vi "[ce] Error Handler.vi"(6 "nesting level":i32, 8 "error in":errorcluster, 9 "error reason":string, 10 "error location":string, 11 "error code":i32) -> (0 "error out":errorcluster, 3 "error":bool)   [LabVIEW 2021]
doc: "The VI builds standard error cluster on the base of input parameters and returns it in <B>error out</B> cluster. If <B>error in</B> indicates an error or <B>error code</B> is zero, <B>error out</B> returns the same value as <B>error in</B>.\n\nIf <B>error code</B> is not zero, the VI puts its value to the <B>code</B> member of the <B>error out</B> cluster and sets the <B>status</B> member to TRUE.\n\n<B>error location</B> specifies location information of an error. If it is empty string, the VI adds VI names in a call chain to this VI. Herewith, <B>nesting level</B> allows to discard VI names at the end of call chain; e.g. zero value discards name of this VI, value of 1 discards name of this VI and name of its caller, and so on. Error location information is put to the <B>source</B> member of the <B>error out</B> cluster.\n\nIf <B>error reson</B> is not empty string, it is added to the <B>source</B> member of the <B>error out</B> cluster.\n\n::: CalcExpress Toolkit :::\nCopyright (c) 2000-2026 Konstantin Shifershteyn. All rights reserved."
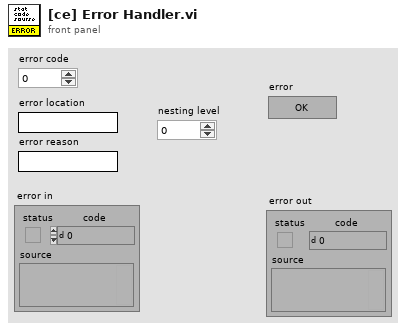
[diagram p1: front panel]
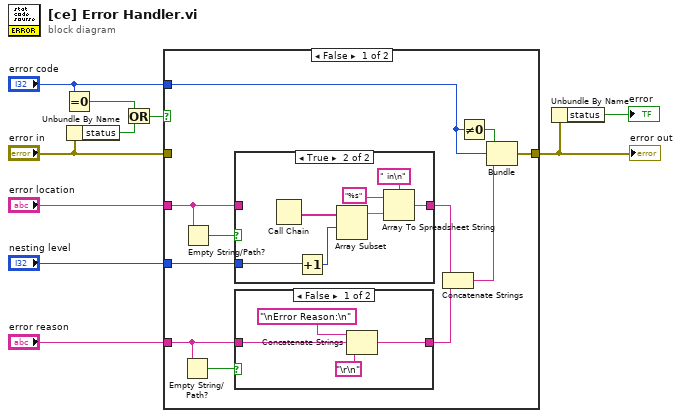
[diagram p0: block diagram]
diagram:
  n1 = Equal To 0?(x="error code") -> (x = 0?=w9:bool)
  n2 = Unbundle By Name("error in") -> ("status"=w10:bool)
  n3 = Or(x=w9, y=w10) -> (x .or. y?=w6:bool)
  n4 = case shown="False" w6 {
    tunnel: "error code" -> [w19 _]
    tunnel: "error in" -> [_ w35]
    tunnel: [w20 w35] -> w4
    tunnel: "error location" -> [w13 _]
    tunnel: "error reason" -> [w12 _]
    tunnel: "nesting level" -> [w11 _]
    frame False {
      n5 = Empty String/Path?(string/path=w12) -> (empty?=w17:bool)
      n6 = Empty String/Path?(string/path=w13) -> (empty?=w21:bool)
      n7 = case shown="True" w21 {
        tunnel: w13 -> [w27 _]
        tunnel: [w27 w29] -> w16
        tunnel: w11 -> [_ w28]
        frame False {
        }
        frame True {
          n8 = Call Chain() -> (call chain=w33:string[])
          n9 = Increment(x=w28) -> (x+1=w34:i32)
          n10 = Array Subset(array=w33, index=w34) -> (w32:string[])  [unwired: 1 in]
          n11 = Array To Spreadsheet String(delimiter (Tab)=" in\n", array=w32, 3:"%s" ("format string")) -> (spreadsheet string=w29:string)
        }
      }
      n12 = case shown="False" w17 {
        tunnel: w12 -> [w23 w26]
        tunnel: [w22 w26] -> w15
        frame False {
          n13 = Concatenate Strings("\nError Reason:\n", w23, "\r\n" ("End of Line Constant")) -> (w22:string)
        }
        frame True {
        }
      }
      n14 = Concatenate Strings(w16, w15) -> (w14:string)
      n15 = Not Equal To 0?(x=w19) -> (x != 0?=w18:bool)
      n16 = Bundle(w18, "error code"=w19, w14) -> (w20:cluster{bool, "error code":i32, string})  [unwired: 1 in]
    }
    frame True {
    }
  }
  "error out" <- w4
  n17 = Unbundle By Name(w4) -> ("status"=→"error":bool)
